vi "Write Control Text.vi"(8 "error in (no error)":errorcluster, 9 "True Text":string, 10 "False Text":string, 11 "Control in":refnum<class "Control.lvclass">) -> (0 "error out":errorcluster, 3 "Control out":refnum<class "Control.lvclass">)   [LabVIEW 2012, in "Control.lvclass"]
doc: "Accessor VI for the control class"
uses:
  Control.lvclass
  Control.lvclass/Control.ctl
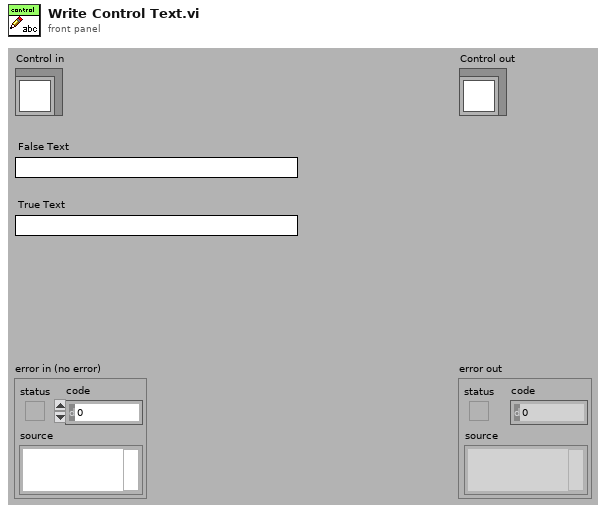
[diagram p1: front panel]
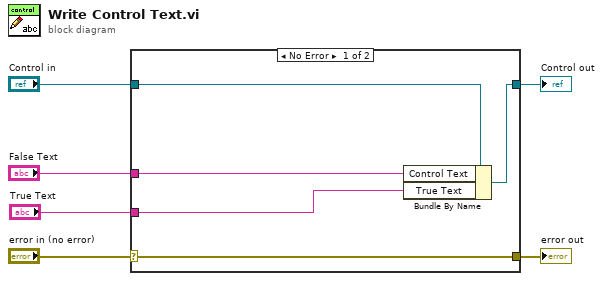
[diagram p0: block diagram]
diagram:
  n1 = case shown="No Error" "error in (no error)" {
    selector: "error in (no error)" -> [w11 w12]
    tunnel: [w11 w12] -> w5
    tunnel: [w9 w13] -> w3
    tunnel: "Control in" -> [w10 w13]
    tunnel: "False Text" -> [w8 _]
    tunnel: "True Text" -> [w7 _]
    frame No Error {
      n2 = Bundle By Name(cluster=w10, "Control Text"=w8, "True Text"=w7) -> (w9:refnum<class "Control.lvclass">)
    }
    frame Error {
    }
  }
  "error out" <- w5
  "Control out" <- w3
